vi "Grab LabVIEW Versions.vi"() -> (2 "Selection":string, 3 "Strings and Values":cluster{"string":string, "value":string}[](array[cluster]))   [LabVIEW 2021, in "TSC Button Editor.lvclass"]
doc: "See all of the available versions to save the button for compatiblity.\n\n<b>Code Developed By:</b> +\nDaniel Coons +\nTechnology Service Corporation +\nwww.tsc.com/atcs"
uses:
  TSC Button Editor.lvclass
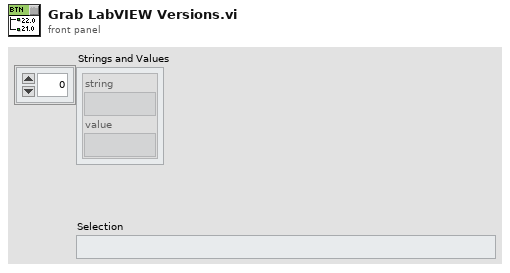
[diagram p1: front panel]
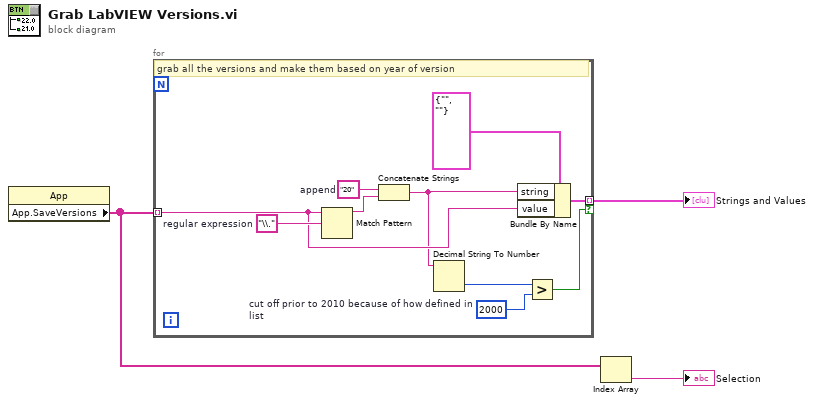
[diagram p0: block diagram]
diagram:
  n1 = property class="App"() -> ("App.SaveVersions"=w3:string[])  [unwired: 2 in, 2 out]
  n2 = for {
    tunnel: w3 -> [w9] mode=indexing
    tunnel: [w8] -> w2 mode=indexing if=w4
    w5 = 2000  # cut off prior to 2010 because of how defined in list
    w11 = "20"  # append
    w13 = "\\."  # regular expression
    # "grab all the versions and make them based on year of version"
    n3 = Match Pattern(string=w9, regular expression=w13) -> (before substring=w12:string)  [unwired: 1 in, 3 out]
    n4 = Concatenate Strings(w11, w12) -> (w7:string)
    n5 = Decimal String To Number(string=w7) -> (number=w6:i32)  [unwired: 2 in, 1 out]
    n6 = Bundle By Name(cluster=cluster{"string":string, "value":string} {"string"="", "value"=""}, "string"=w7, "value"=w9) -> (w8:cluster{"string":string, "value":string})
    n7 = Greater?(x=w6, y=w5) -> (0:w4:bool)
  }
  "Strings and Values" <- w2
  n8 = Index Array(array=w3) -> (element=→"Selection":string)  [unwired: 1 in]
